vi "Blue--constant.vi"() -> (1 "Blue":u32(colorbox))   [LabVIEW 2018, in "Band Colors.lvlib"]
doc: "Provides the RGB color value for blue.\n\nThe VI converts the RGB components (0, 70, 220) into a LabVIEW color value and returns it through <b>Blue</b>."
uses:
  Band Colors.lvlib
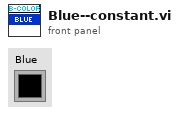
[diagram p1: front panel]
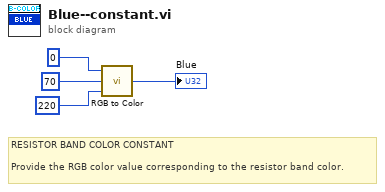
[diagram p0: block diagram]
diagram:
  # "RESISTOR BAND COLOR CONSTANT\n\nProvide the RGB color value corresponding to the resistor band color."
  n1 = call <vilib>:"RGB to Color.vi"("B"=u8 220, "G"=u8 70, "R"=u8 0) -> ("Color"=→"Blue":u32)
